vi "Generate Results.vi"(8 "error in (no error)":errorcluster, 10 "Storage":refnum<class "Test Event Storage.lvclass">, 11 "Basic Test Manager in":refnum<class "Basic Test Manager.lvclass">) -> (0 "error out":errorcluster, 2 "Test Result":refnum<class "Test Result.lvclass">, 3 "Basic Test Manager out":refnum<class "Basic Test Manager.lvclass">)   [LabVIEW 2020, in "Caraya.lvlib" / "Basic Test Manager.lvclass"]
uses:
  Basic Test Manager.lvclass
  Test Event Storage/Test Event Storage.lvclass
  Test Result/Test Result.lvclass
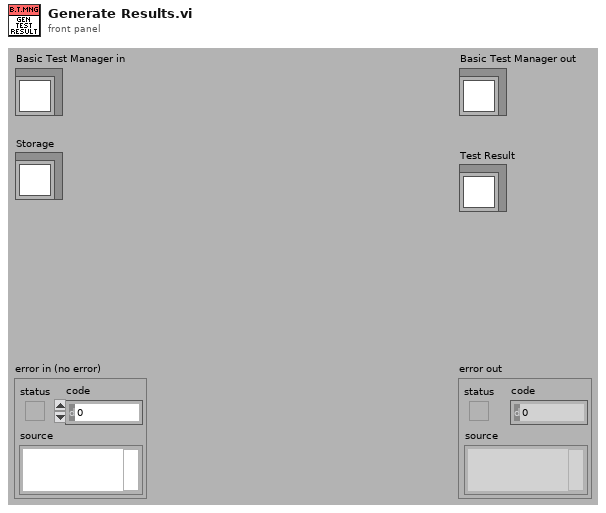
[diagram p1: front panel]
types:
  T1 = typedef "Caraya.lvlib/Test Result.lvclass/Test Node (Extended).ctl" = cluster{"Test Registration":T2, "Defined":bool, "Passed":bool, "properties":variant}
  T2 = typedef "Caraya.lvlib/Test Result.lvclass/Test Registration Data.ctl" = cluster{"Name":string, "Call Chain":string[], "Time Stamp":timestamp, "Test ID":string, "Caller ID":string}
  T3 = typedef "Caraya.lvlib/Test Result.lvclass/Assert Event Data (Extended).ctl" = cluster{"name":string, "passed":bool, "call-chain":string[], "test-error":errorcluster, "timestamp":timestamp, "assert-id":string, "test-id":string, "time":dbl, "message":string, "properties":variant, "measurements":variant, "user-defined":variant}
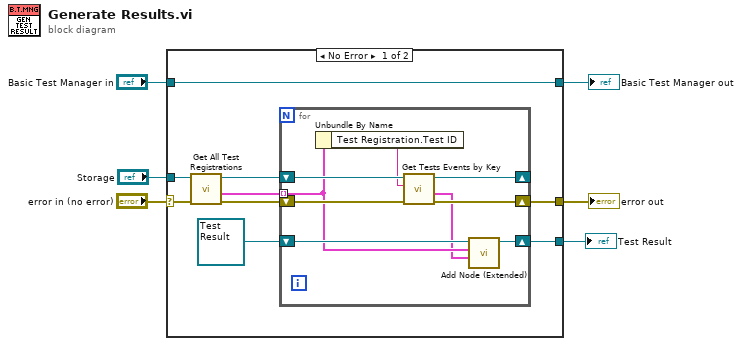
[diagram p0: block diagram]
diagram:
  n1 = case shown="No Error" "error in (no error)" {
    selector: "error in (no error)" -> [w13 w26]
    tunnel: [w11 w26] -> w5
    tunnel: [w8 w25] -> w3
    tunnel: "Basic Test Manager in" -> [w8 w25]
    tunnel: "Storage" -> [w15 _]
    tunnel: [w10 _] -> w1
    frame No Error {
      n2 = call-dynamic "Get All Test Registrations.vi"("error in (no error)"=w13, "Test Event Storage in"=w15) -> ("error out"=w12:errorcluster, "Test Registrations"=w7:T1[], "Test Event Storage out"=w14:refnum<class "Test Event Storage.lvclass">)  [unwired: 5 in, 2 out]
      n3 = for {
        tunnel: w7 -> [w18] mode=indexing
        shift-right: [w16] -> w10
        shift-left: refnum<class "Test Result.lvclass"> refnum ("Caraya.lvlib:Test Result.lvclass") -> [w19]
        shift-right: [w23] -> _
        shift-left: w14 -> [w24]
        shift-right: [w21] -> w11
        shift-left: w12 -> [w22]
        n4 = Unbundle By Name(w18) -> ("Test Registration.Test ID"=w20:string)
        n5 = call "Get Tests Events by Key.vi"("error in (no error)"=w22, "Key (Test ID)"=w20, "Test Event Storage in"=w24) -> ("error out"=w21:errorcluster, "Assertions"=w17:T3[], "Test Event Storage out"=w23:refnum<class "Test Event Storage.lvclass">)  [unwired: 6 in]
        n6 = call "Add Node (Extended).vi"("Assertions"=w17, "Test Node"=w18, "Test Result in"=w19) -> ("Test Result out"=w16:refnum<class "Test Result.lvclass">)  [unwired: 7 in, 1 out]
      }
    }
    frame Error {
    }
  }
  "error out" <- w5
  "Basic Test Manager out" <- w3
  "Test Result" <- w1
